vi "Write Outputs2.vi"(8 "error in (no error)":errorcluster, 10 "Analog Outputs":sgl[](array[numeric]), 11 "M5StackDAC2 in":refnum<class "M5StackDAC2.lvclass">) -> (0 "error out":errorcluster, 3 "M5StackDAC2 out":refnum<class "M5StackDAC2.lvclass">)   [LabVIEW 2020]
uses:
  M5StackDAC2.lvclass/M5StackDAC2.ctl
  CTI/I2C Connection/I2C Connection.lvclass
  M5StackDAC2.lvclass
  C:/Users/Public/SourceGit/cti-drivers-lv-visa/CTI-Peripheral/Analog Output/Grove An Out/M5StackDAC2/M5StackDAC2.lvclass
  C:/Users/Public/SourceGit/cti-drivers-lv-visa/CTI-Peripheral/Analog Output/Grove An Out/Base/An Out I2C.lvclass
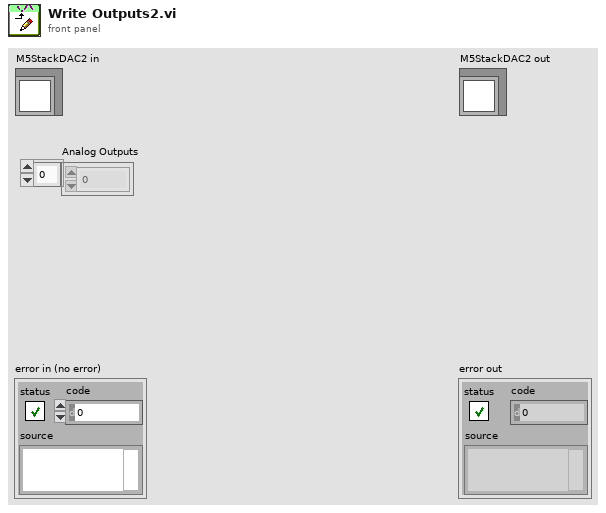
[diagram p1: front panel]
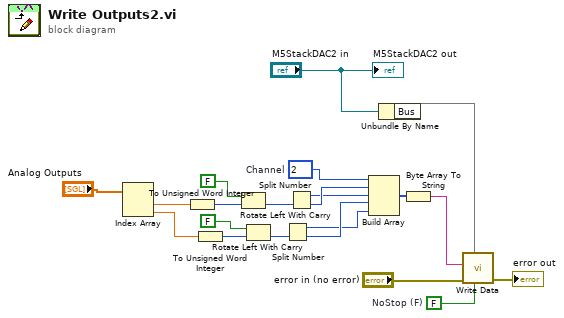
[diagram p0: block diagram]
diagram:
  w17 = u8 2  # Channel
  w18 = FALSE  # NoStop (F)
  n1 = Index Array(array="Analog Outputs") -> (element #1=w4:sgl, element #2=w3:sgl)  [unwired: 2 in]
  n2 = To Unsigned Word Integer(number=w4) -> (unsigned 16bit integer=w2:u16)
  n3 = To Unsigned Word Integer(number=w3) -> (unsigned 16bit integer=w1:u16)
  n4 = Rotate Left With Carry(2:w2, 3:FALSE ("carry")) -> (0:w15:u16)  [unwired: 1 out]
  n5 = Rotate Left With Carry(2:w1, 3:FALSE ("carry")) -> (0:w13:u16)  [unwired: 1 out]
  n6 = Split Number(x=w13) -> (hi(x)=w9:u8, lo(x)=w10:u8)
  n7 = Split Number(x=w15) -> (hi(x)=w11:u8, lo(x)=w12:u8)
  n8 = Build Array(w17, w12, w11, w10, w9) -> (w8:u8[])
  n9 = Unbundle By Name("M5StackDAC2 in") -> ("Bus"=w19)
  n10 = Byte Array To String(unsigned byte array=w8) -> (string=w6:string)
  n11 = call "Write Data.vi"("NoStop (F)"=w18, "I2C Connection"=w19, "error in (no error)"="error in (no error)", "Data"=w6) -> ("error out"=→"error out":errorcluster)  [unwired: 7 in]
  "M5StackDAC2 out" <- "M5StackDAC2 in"
